vi "Init.vi"(8 "error in (no error)":errorcluster, 10 "Last Update (Current)":timestamp, 11 "Path":path) -> (0 "error out":errorcluster, 3 "ViaApp out":refnum<class "ViaApp.lvclass">)   [LabVIEW 2020, in "PicoG-App.lvlib" / "ViaApp.lvclass"]
uses:
  ViaApp.lvclass
  ViaApp.lvclass/ViaApp.ctl
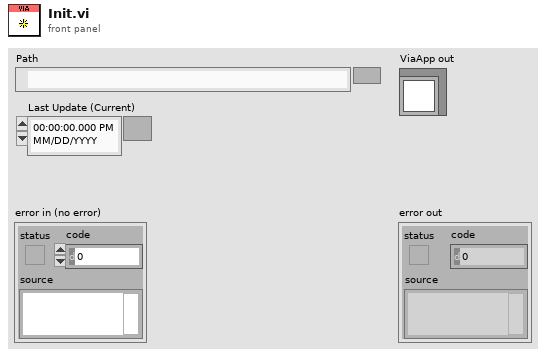
[diagram p1: front panel]
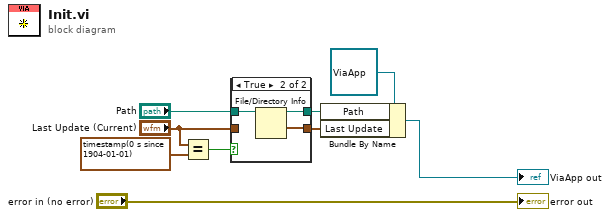
[diagram p0: block diagram]
diagram:
  n1 = Equal?(x="Last Update (Current)", y=timestamp(0 s since 1904-01-01) ("Last Update (None)")) -> (x = y?=w5:bool)
  n2 = case shown="True" w5 {
    tunnel: "Last Update (Current)" -> [w11 _]
    tunnel: "Path" -> [w10 w14]
    tunnel: [w10 w13] -> w2
    tunnel: [w11 w12] -> w1
    frame False {
    }
    frame True {
      n3 = File/Directory Info(path=w14) -> (path out=w13:path, last mod=w12:timestamp)  [unwired: 1 in, 5 out]
    }
  }
  n4 = Bundle By Name(cluster=refnum<class "ViaApp.lvclass"> refnum ("ViaApp in"), "Path"=w2, "Last Update"=w1) -> (→"ViaApp out":refnum<class "ViaApp.lvclass">)
  "error out" <- "error in (no error)"
